vi "Main1.vi"(10 "Test Titel":string, 11 "Cluster 2":T1={"Test Titel"="", "Test Type "="", "Project Number"="NA", "Unit Family"="Package", "Test Procedure #"="", "Data Collection Rate (HZ)"="", "Cluster"={" Pressure /Torque/ LVDT"={"Boolean"=FALSE, "Boolean 2"=FALSE, "Boolean 3"=FALSE, "Boolean 4"=FALSE, "Boolean 5"=FALSE, "Boolean 6"=FALSE, "Boolean 7"=FALSE, "Boolean 8"=FALSE}, "Name of Channel"={"ch1"="", "ch1 2"="", "ch1 3"="", "ch1 4"="", "ch1 5"="", "ch1 6"="", "ch1 7"="", "ch1 8"=""}, "Create New Test"=FALSE, "Name of Channel 2"={"ch1"="", "ch1 2"="", "ch1 3"="", "ch1 4"="", "ch1 5"="", "ch1 6"="", "ch1 7"="", "ch1 8"="", "ch1 9"="", "ch1 10"="", "ch1 11"="", "ch1 12"="", "ch1 13"="", "ch1 14"="", "ch1 15"=""}, "MOD1 ThermoCouple"={"Boolean"=FALSE, "Boolean 2"=FALSE, "Boolean 3"=FALSE, "Boolean 4"=FALSE, "Boolean 5"=FALSE, "Boolean 6"=FALSE, "Boolean 7"=FALSE, "Boolean 8"=FALSE, "Boolean 9"=FALSE, "Boolean 10"=FALSE, "Boolean 11"=FALSE, "Boolean 12"=FALSE, "Boolean 13"=FALSE, "Boolean 14"=FALSE, "Boolean 15"=FALSE, "Boolean 16"=FALSE}, "Internal SFI sensor number"={"ch1"="", "ch1 2"="", "ch1 3"="", "ch1 4"="", "ch1 5"="", "ch1 6"="", "ch1 7"="", "ch1 8"=""}, "Internal SFI sensor number"={"ch1"="", "ch1 2"="", "ch1 3"="", "ch1 4"="", "ch1 5"="", "ch1 6"="", "ch1 7"="", "ch1 8"="", "ch1 9"="", "ch1 10"="", "ch1 11"="", "ch1 12"="", "ch1 13"="", "ch1 14"="", "ch1 15"=""}}, "Sensor Serial Num"="", "Calibration Due"=""}) -> (3 "Waveform Graph":dbl[][](graph))   [LabVIEW 2024]
uses:
  States.ctl
  Global 1.vi
  Wave forms.vi
panel:
  out "appended array 3":dbl[](array[numeric])
  in  "Table Control":string[][](table)
  out "Symbol":string
  in  "Combo Box":string(combo)
  in  "Boolean 2":bool
  in  "Log Interval\n(seconds)":dbl=0.5 min=0.1 max=10.0 step=0.1
  in  "Hours to Show 2":dbl=0.05
  in  "stop":bool
  out "appended array":string[](array[string])
  out "Array 3":string[](array[string])
  out "Array 2":string[](array[string])
  in  "Array":dbl[](array[numeric])
  in  "Boolean":bool
  out "Last Event Time (sec)":i32
  out "Event Counter":i32
  in  "Tab Control":enum32{"Main Configuration", "Graphs Display"}(tab)
  in  "End pro":bool
  in  "Settings Button":bool
  in  "Add paramter":bool
  in  "Select Parameter to ADD":string(combo)
  in  "Record Button":bool
  in  "end":bool caption="Pause Button 2"
  in  "Initial":bool caption="Pause Button"
  in  "Start Test":bool caption="OK Button"
  # "Valves Testing System"
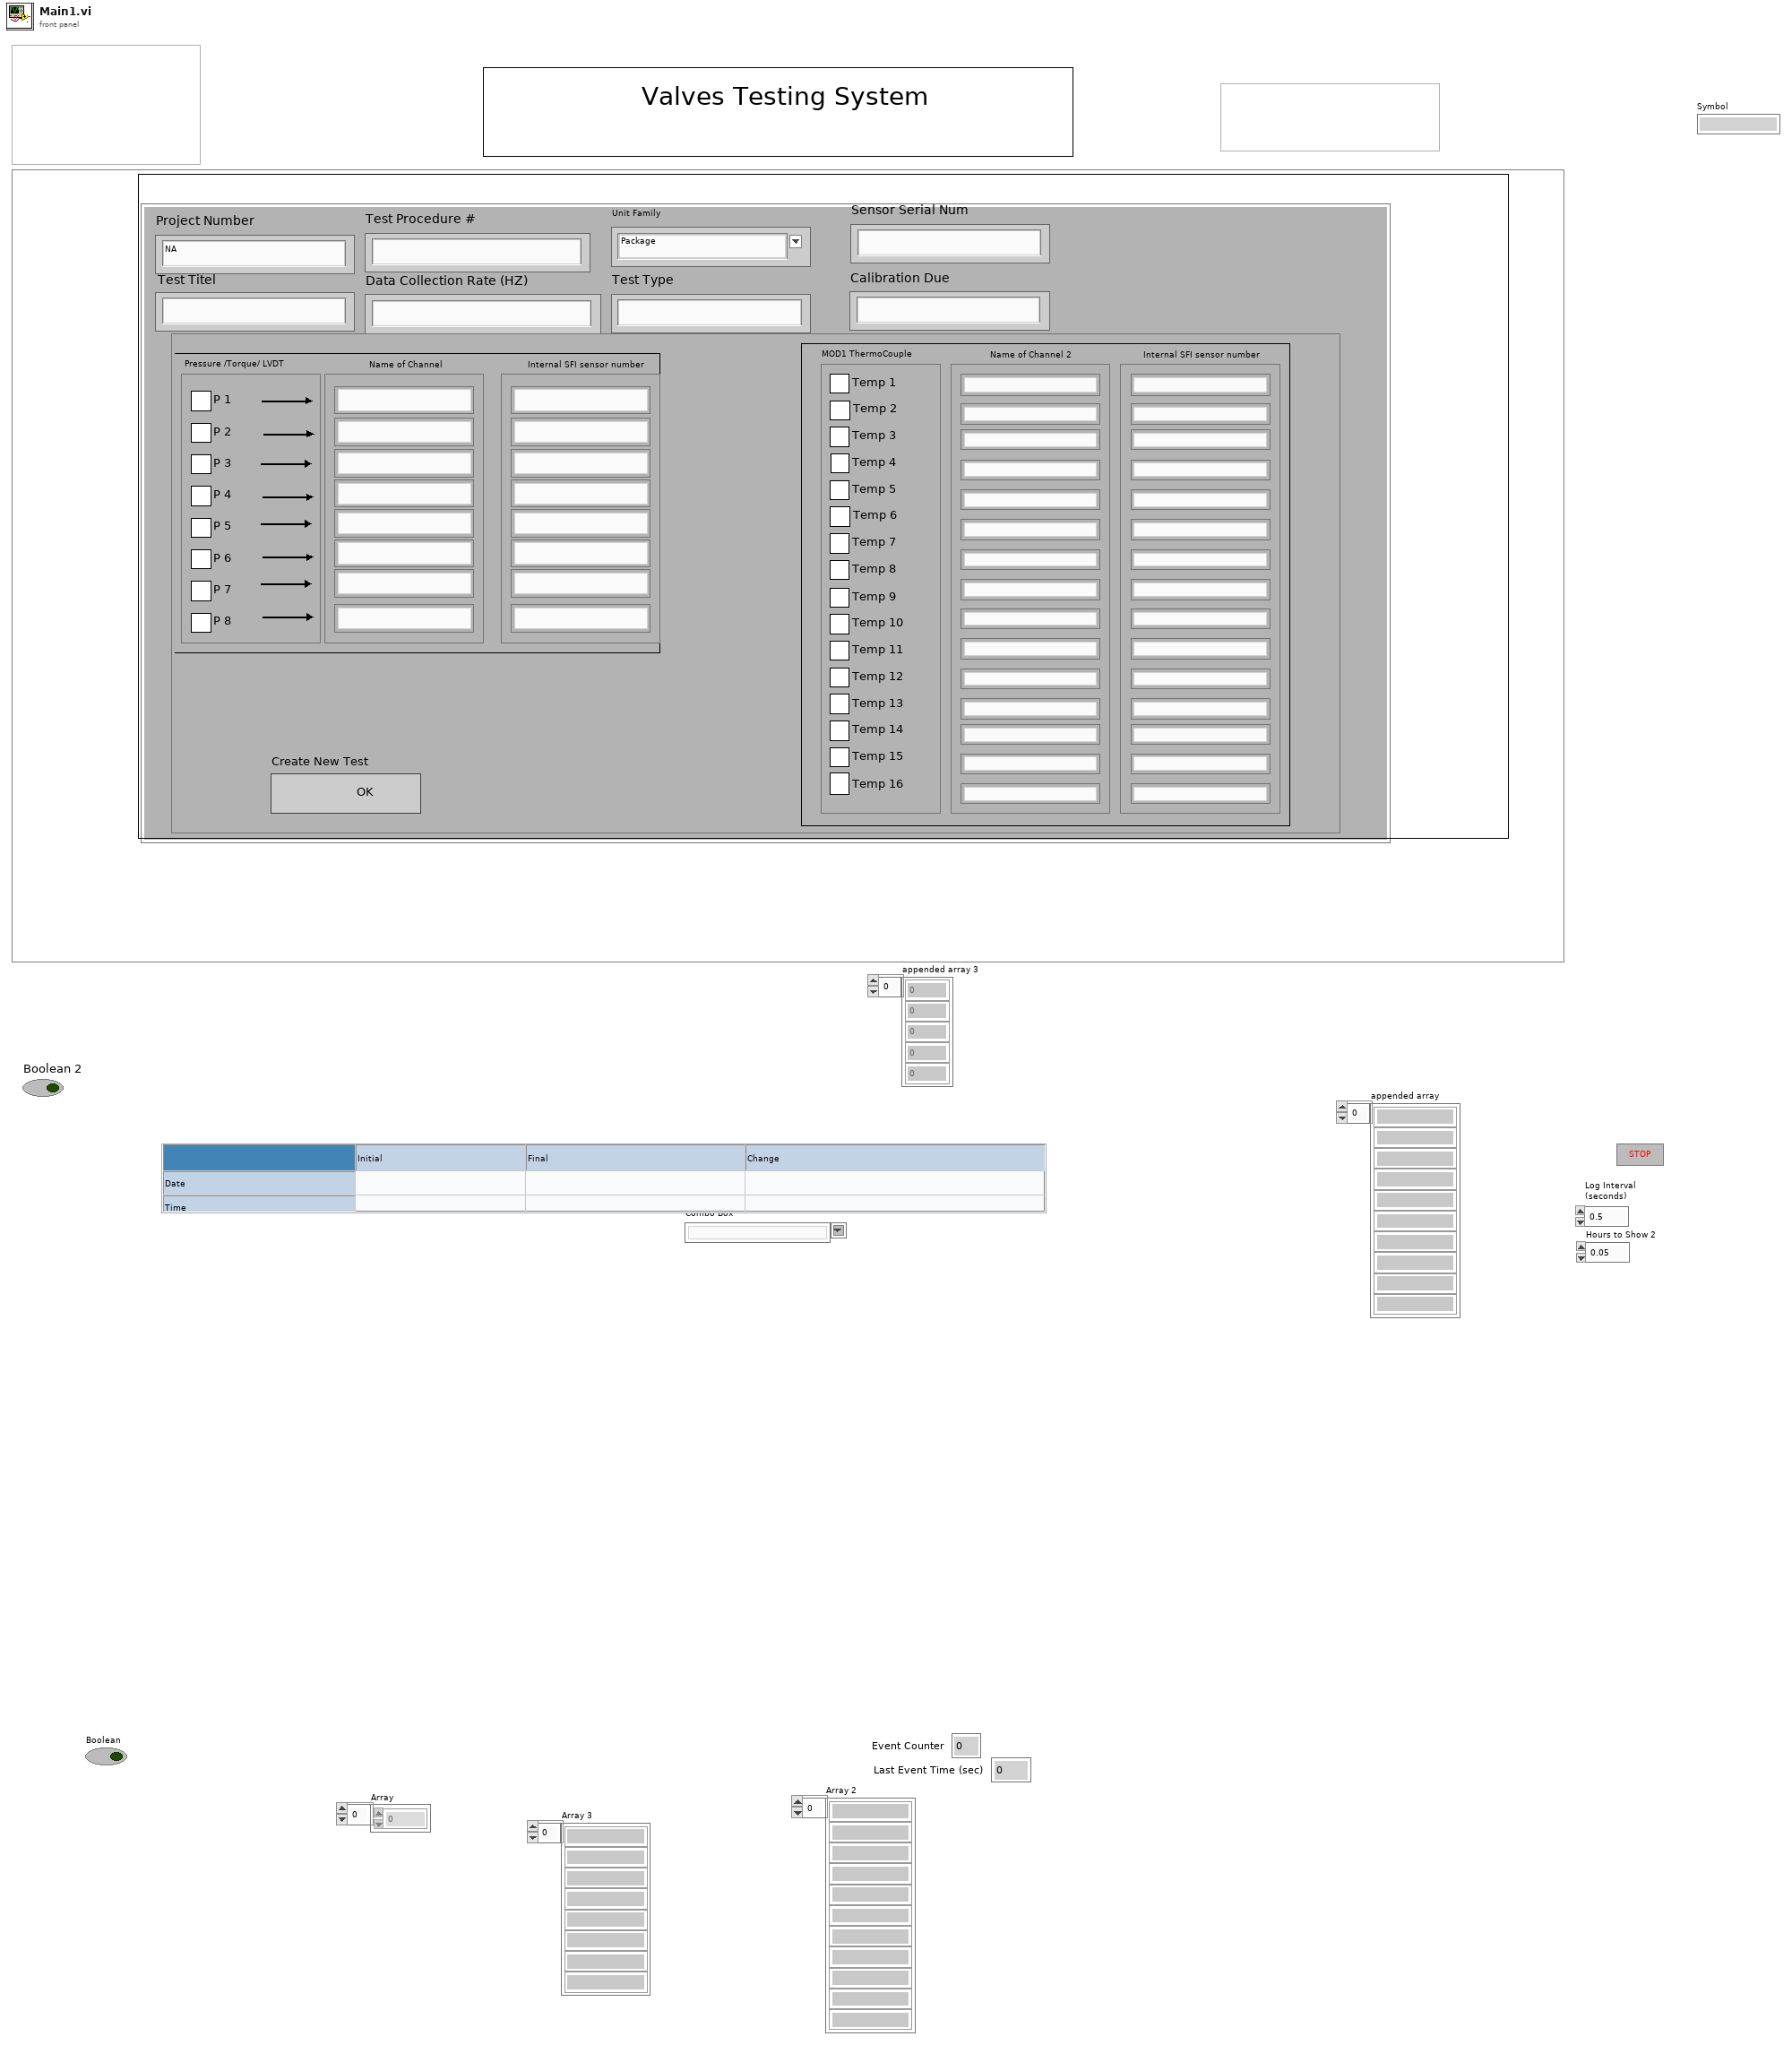
[diagram p1: front panel]
types:
  T1 = cluster{"Test Titel":string, "Test Type ":string, "Project Number":string, "Unit Family":string, "Test Procedure #":string, "Data Collection Rate (HZ)":string, "Cluster":cluster{" Pressure /Torque/ LVDT":cluster{"Boolean":bool, "Boolean 2":bool, "Boolean 3":bool, "Boolean 4":bool, "Boolean 5":bool, "Boolean 6":bool, "Boolean 7":bool, "Boolean 8":bool}, "Name of Channel":cluster{"ch1":string, "ch1 2":string, "ch1 3":string, "ch1 4":string, "ch1 5":string, "ch1 6":string, "ch1 7":string, "ch1 8":string}, "Create New Test":bool, "Name of Channel 2":cluster{"ch1":string, "ch1 2":string, "ch1 3":string, "ch1 4":string, "ch1 5":string, "ch1 6":string, "ch1 7":string, "ch1 8":string, "ch1 9":string, "ch1 10":string, "ch1 11":string, "ch1 12":string, "ch1 13":string, "ch1 14":string, "ch1 15":string}, "MOD1 ThermoCouple":cluster{"Boolean":bool, "Boolean 2":bool, "Boolean 3":bool, "Boolean 4":bool, "Boolean 5":bool, "Boolean 6":bool, "Boolean 7":bool, "Boolean 8":bool, "Boolean 9":bool, "Boolean 10":bool, "Boolean 11":bool, "Boolean 12":bool, "Boolean 13":bool, "Boolean 14":bool, "Boolean 15":bool, "Boolean 16":bool}, "Internal SFI sensor number":cluster{"ch1":string, "ch1 2":string, "ch1 3":string, "ch1 4":string, "ch1 5":string, "ch1 6":string, "ch1 7":string, "ch1 8":string}, "Internal SFI sensor number":cluster{"ch1":string, "ch1 2":string, "ch1 3":string, "ch1 4":string, "ch1 5":string, "ch1 6":string, "ch1 7":string, "ch1 8":string, "ch1 9":string, "ch1 10":string, "ch1 11":string, "ch1 12":string, "ch1 13":string, "ch1 14":string, "ch1 15":string}}, "Sensor Serial Num":string, "Calibration Due":string}
  T2 = typedef "States.ctl" = enum16{"Idel", "end test", "Selection", "Inittialize"}
  T3 = cluster{"Paramter":string, "Intital ":string, "Final":string, "Change":string, "Alarm Activate ":bool, "Symbol":string, "Value":string, "Alarm":bool}[]
  T4 = cluster{"Paramter":string, "Rate of Change":dbl, "X (sec)":dbl}[]
  T5 = cluster{"Paramter":string, "Intital ":string, "Final":string, "Change":string, "Alarm Activate ":bool, "Symbol":string, "Value":string, "Alarm":bool}
  T6 = cluster{"ch1":string, "ch1 2":string, "ch1 3":string, "ch1 4":string, "ch1 5":string, "ch1 6":string, "ch1 7":string, "ch1 8":string, "ch1 9":string, "ch1 10":string, "ch1 11":string, "ch1 12":string, "ch1 13":string, "ch1 14":string, "ch1 15":string}
  T7 = cluster{"Boolean":bool, "Boolean 2":bool, "Boolean 3":bool, "Boolean 4":bool, "Boolean 5":bool, "Boolean 6":bool, "Boolean 7":bool, "Boolean 8":bool, "Boolean 9":bool, "Boolean 10":bool, "Boolean 11":bool, "Boolean 12":bool, "Boolean 13":bool, "Boolean 14":bool, "Boolean 15":bool, "Boolean 16":bool}
  T8 = cluster{"Boolean":bool, "Boolean 2":bool, "Boolean 3":bool, "Boolean 4":bool, "Boolean 5":bool, "Boolean 6":bool, "Boolean 7":bool, "Boolean 8":bool}
  T9 = cluster{"ch1":string, "ch1 2":string, "ch1 3":string, "ch1 4":string, "ch1 5":string, "ch1 6":string, "ch1 7":string, "ch1 8":string}
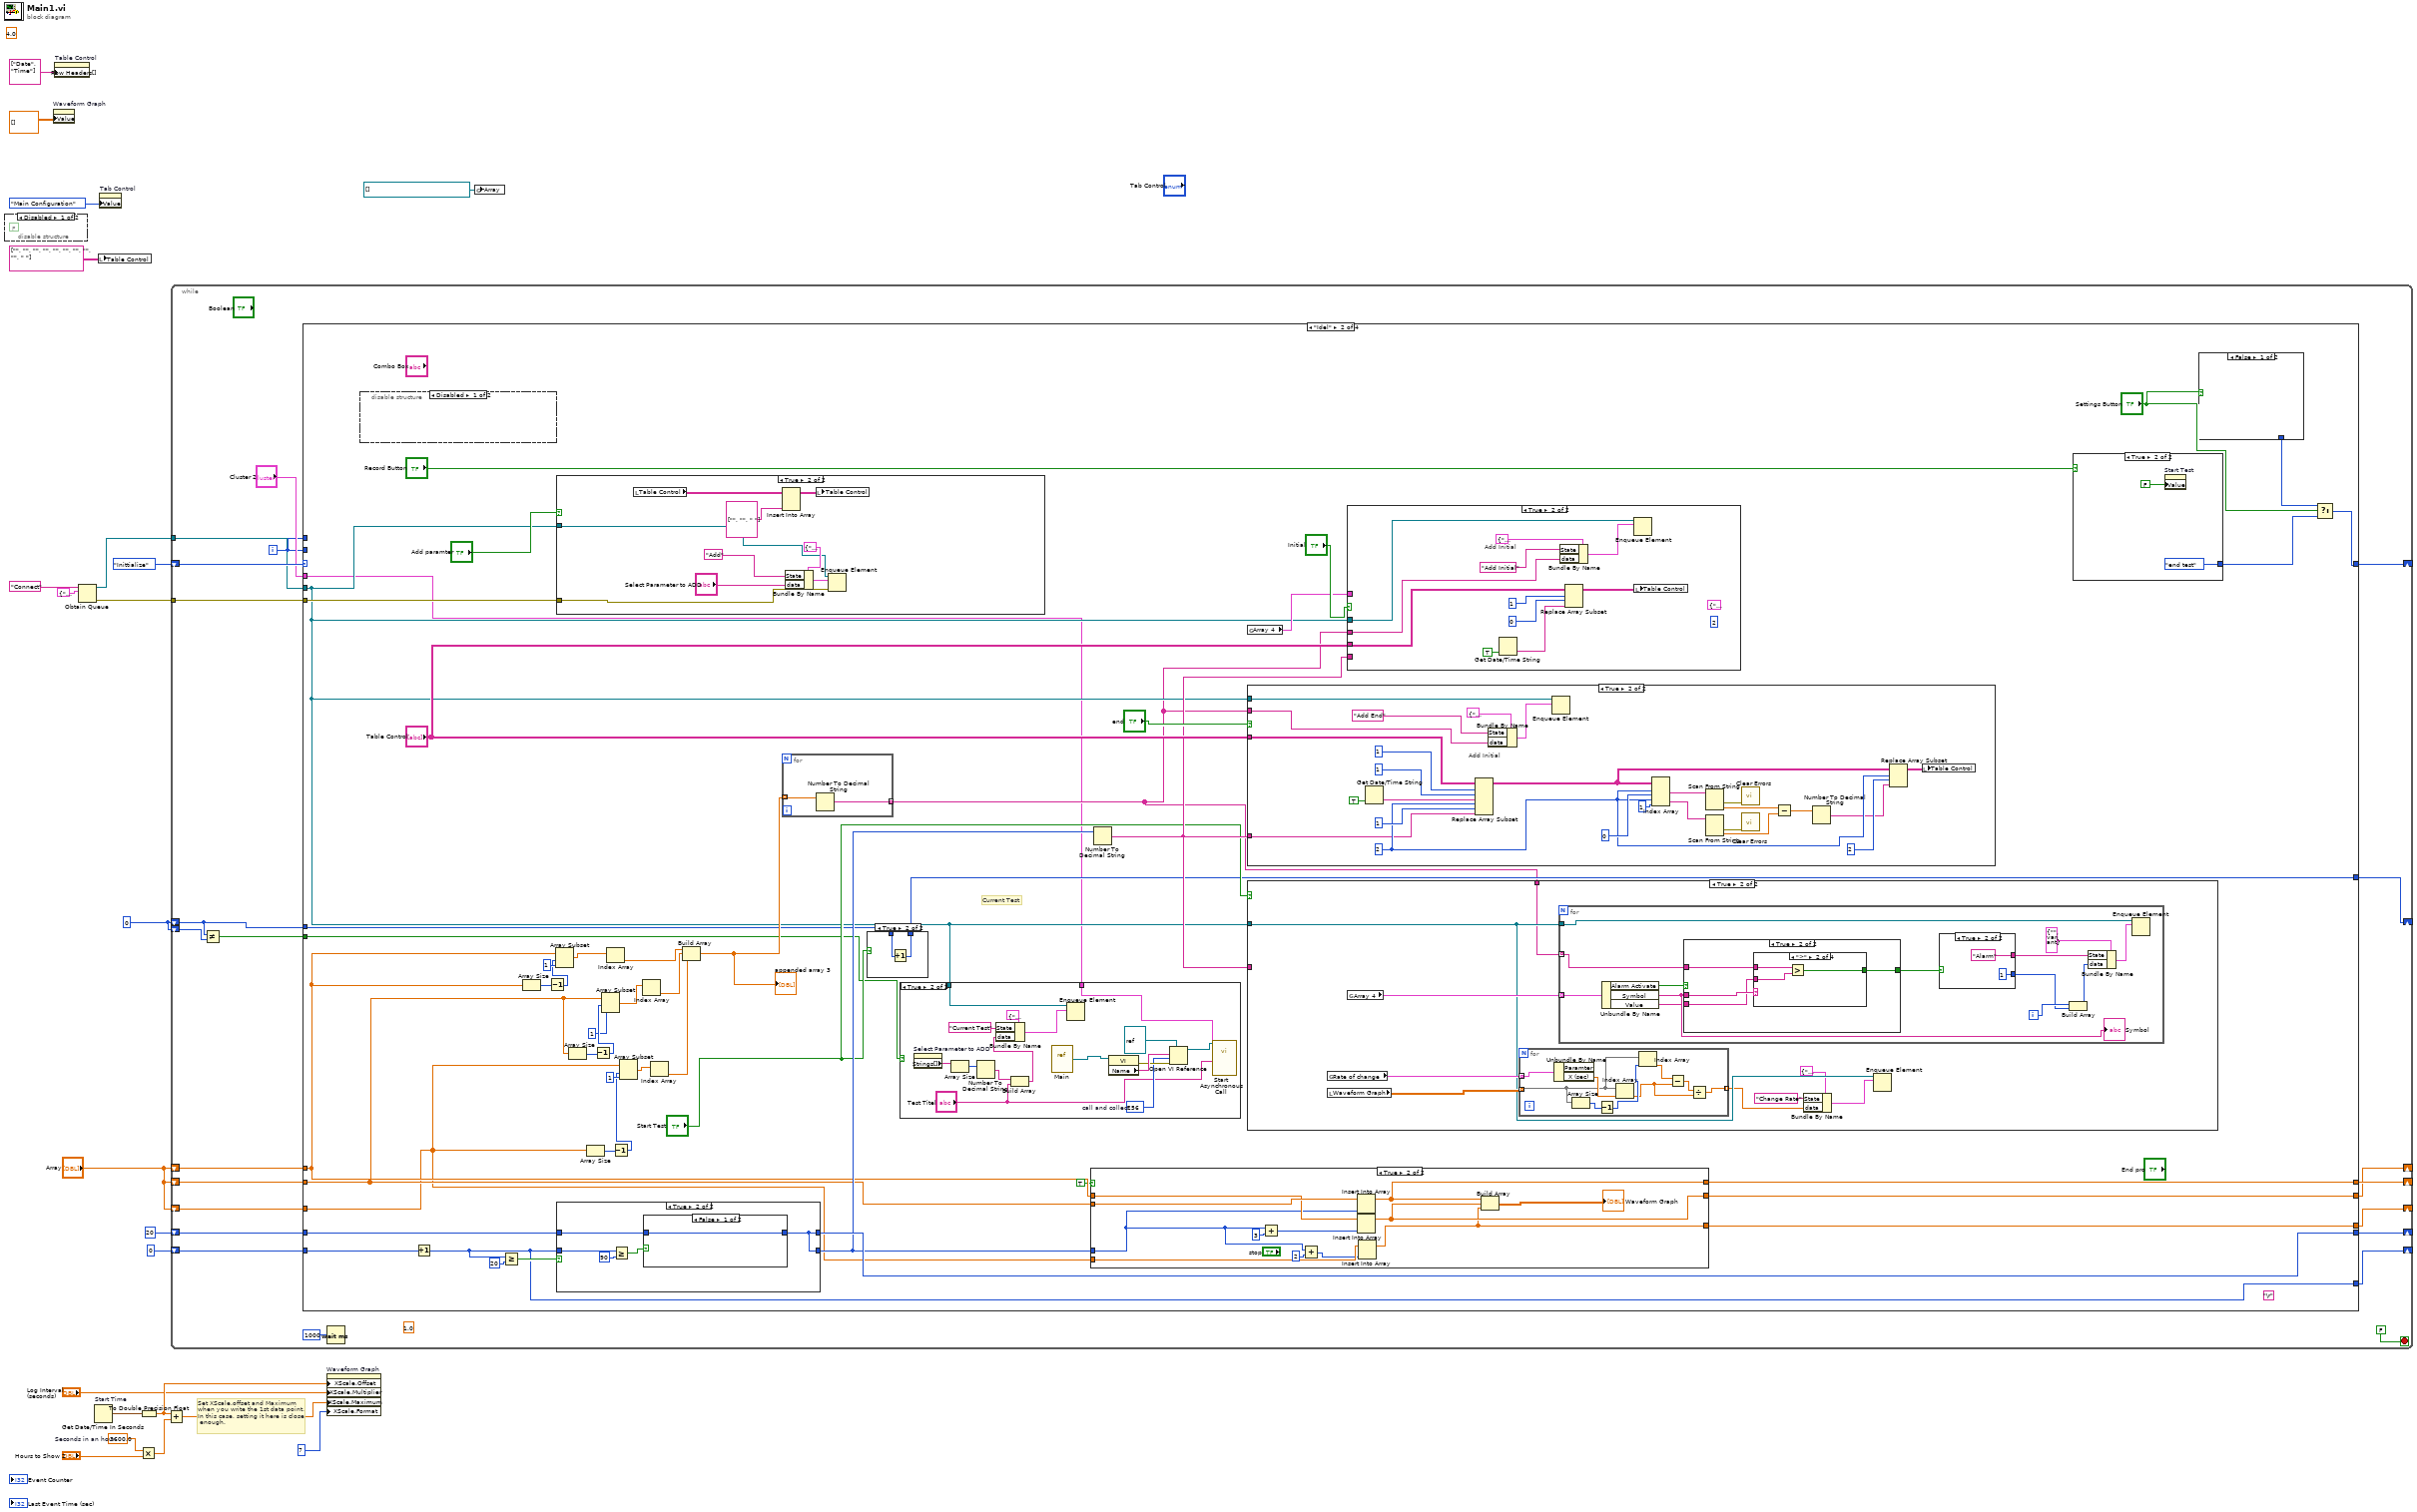
[diagram p0: block diagram]
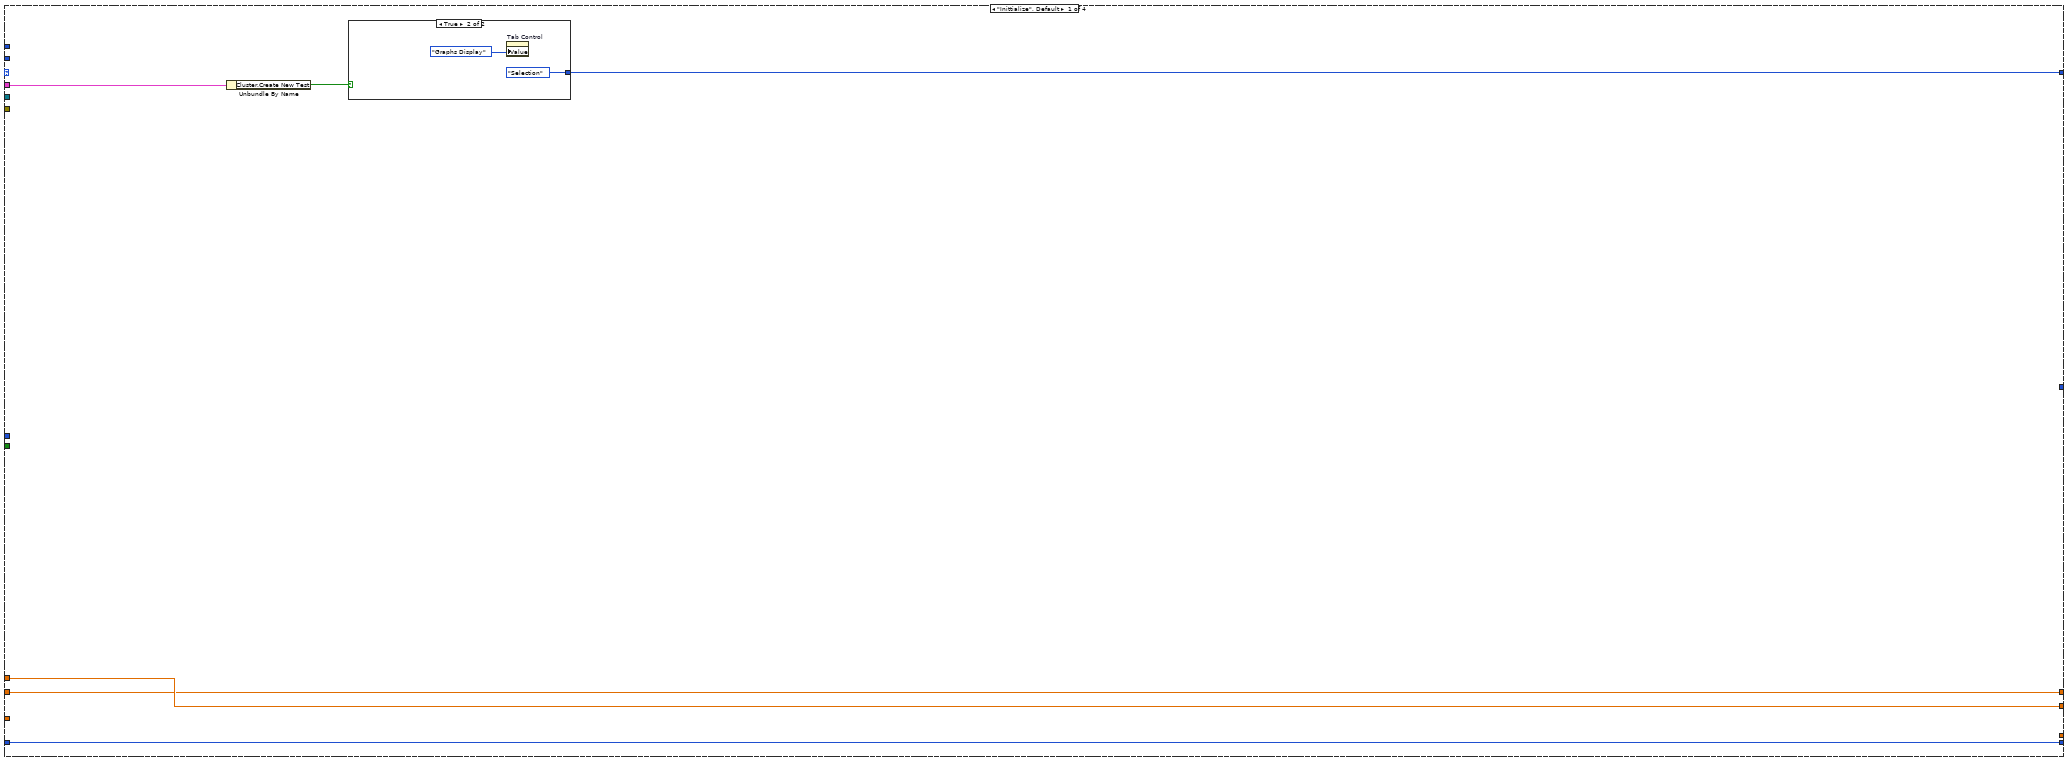
[diagram p3: hidden frame]
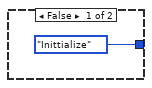
[diagram p4: hidden frame]
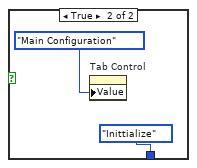
[diagram p7: hidden frame]
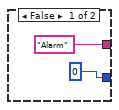
[diagram p9: hidden frame]
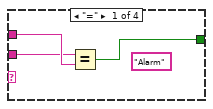
[diagram p11: hidden frame]
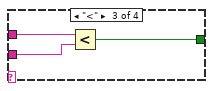
[diagram p12: hidden frame]
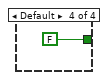
[diagram p13: hidden frame]
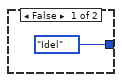
[diagram p15: hidden frame]
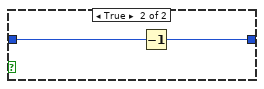
[diagram p20: hidden frame]
diagram:
  w2 = 0
  (unwired) 4.0
  w18 = 3600.0  # Seconds in an hour
  # "Set XScale.offset and Maximum\nwhen you write the 1st data point. \nIn this case, setting it here is close\n enough."
  n1 = disable-structure shown="Disabled" {
    frame Disabled {
      (unwired) FALSE ("OK Button")
    }
    frame Enabled {
    }
  }
  n2 = property on="Waveform Graph" class="WFGraph (strict)"("Value"=dbl[][] [] ("Waveform Graph")) -> ()  [unwired: 2 in, 2 out]
  n3 = property on="Table Control" class="Tbl (strict)"("Row Headers[]"=string[] ["Date", "Time"] ("Row Header Strings[]")) -> ()  [unwired: 2 in, 2 out]
  n4 = Obtain Queue(name (unnamed)="Connect", element data type=cluster{"State":string, "data":variant} {"State"="", "data"=variant}) -> (queue out=w5:refnum<queue>, error out=w4:errorcluster)  [unwired: 3 in, 1 out]
  n5 = Get Date/Time In Seconds "Start Time"() -> (seconds since 1Jan1904=w19:timestamp)
  n6 = local write "Table Control"(string[][] [["", "", "", "", ""], ["", "", "", "", " "]] ("Test Results")) -> ()
  n7 = property on="Tab Control" class="TabCtl (strict)"("Value"=enum32{"Main Configuration", "Graphs Display"}."Main Configuration" ("Tab Control")) -> ()  [unwired: 2 in, 2 out]
  n8 = Multiply(x=w18, y="Hours to Show 2") -> (x*y=w20:dbl)
  n9 = To Double Precision Float(number=w19) -> (double precision float=w13:dbl)
  n10 = Add(x=w13, y=w20) -> (x+y=w11:dbl)
  n11 = while {
    shift-right: [w41] -> _
    shift-left: States."Inittialize" -> [w44]
    shift-right: [w38] -> _
    shift-left: "Array" -> [w39]
    shift-right: [w32] -> _
    shift-left: 20 -> [w36]
    shift-right: [w34] -> _
    shift-left: "Array" -> [w35]
    shift-right: [w31] -> _
    shift-left: 0 -> [w33]
    tunnel: w5 -> [w30]
    tunnel: w4 -> [w29]
    shift-right: [w27] -> _
    shift-left: "Array" -> [w28]
    shift-right: [w23] -> _
    shift-left: w2 -> [w25]
    shift-left: w2 -> [w26]
    i -> [w37]
    stop <- FALSE stop-if-true
    (unwired) 1.0 ("Log Interval\n(seconds)")
    n12 = Not Equal?(x=w25, y=w26) -> (x != y?=w24:bool)
    n13 = case shown="\"Idel\"" w44 {
      tunnel: "Cluster 2" -> [w50 w54 w271 _]
      tunnel: [w47 w83 States."Idel" States."end test"] -> w41
      tunnel: w39 -> [w45 w70 _ _]
      tunnel: w37 -> [_ _ _ _]
      tunnel: [w45 w102 _ _] -> w38
      tunnel: w37 -> [_ _ _ _]
      tunnel: [w49 w98 w260 _] -> w32
      tunnel: w36 -> [w49 w97 w260 _]
      tunnel: w35 -> [w46 w79 _ _]
      tunnel: [w46 w91 _ _] -> w34
      tunnel: w33 -> [_ w90 _ _]
      tunnel: [_ w89 _ _] -> w31
      tunnel: w30 -> [_ w56 _ _]
      tunnel: w29 -> [_ w87 _ _]
      tunnel: w28 -> [_ w69 _ _]
      tunnel: [_ w81 _ _] -> w27
      tunnel: w25 -> [_ w60 _ _]
      tunnel: w24 -> [_ w59 _ _]
      tunnel: [_ w58 _ _] -> w23
      frame "Inittialize", Default {
        n14 = Unbundle By Name(w50) -> ("Cluster.Create New Test"=w48:bool)
        n15 = case shown="True" w48 {
          tunnel: [States."Inittialize" States."Selection"] -> w47
          frame False {
          }
          frame True {
            n16 = property on="Tab Control" class="TabCtl (strict)"("Value"=enum32{"Main Configuration", "Graphs Display"}."Graphs Display" ("Tab Control")) -> ()  [unwired: 2 in, 2 out]
          }
        }
      }
      frame "Idel" {
        (unwired) "\r"
        # "Current Test"
        n17 = disable-structure shown="Disabled" {
          frame Disabled {
          }
          frame Enabled {
          }
        }
        n18 = Increment(x=w90) -> (x+1=w89:i32)
        n19 = Greater Or Equal?(x=w89, y=20) -> (x >= y?=w99:bool)
        n20 = Array Size(array=w79) -> (size(s)=w78:i32)
        n21 = Decrement(x=w78) -> (x-1=w77:i32)
        n22 = Array Subset(array=w79, index=w77, length=1) -> (w68:dbl[])
        n23 = case shown="True" "Add paramter" {
          tunnel: w56 -> [_ w241]
          tunnel: w87 -> [_ w240]
          frame False {
          }
          frame True {
            n24 = local read "Table Control"() -> (w247:string[][])
            n25 = Insert Into Array(array=w247, new element=string[] ["", "", " "] ("new element/subarray")) -> (w246:string[][])  [unwired: 2 in]
            n26 = Bundle By Name(cluster=cluster{"State":string, "data":variant} {"State"="", "data"=variant}, "State"="Add", "data"="Select Parameter to ADD") -> (w244:cluster{"State":string, "data":variant})
            n27 = local write "Table Control"(w246) -> ()
            n28 = Enqueue Element(queue=w241, element=w244, error in (no error)=w240) -> ()  [unwired: 1 in, 3 out]
          }
        }
        n29 = case shown="True" w99 {
          tunnel: [w231 w235] -> w93
          tunnel: w89 -> [w231 w234]
          tunnel: [w230 w235] -> w98
          tunnel: w97 -> [w230 w236]
          frame False {
          }
          frame True {
            n30 = Greater Or Equal?(x=w234, y=90) -> (x >= y?=w232:bool)
            n31 = case shown="False" w232 {
              tunnel: w236 -> [w237 w239]
              tunnel: [w237 w238] -> w235
              frame False {
              }
              frame True {
                n32 = Decrement(x=w239) -> (x-1=w238:i32)
              }
            }
          }
        }
        n33 = Array Size(array=w70) -> (size(s)=w75:i32)
        n34 = Array Size(array=w69) -> (size(s)=w72:i32)
        n35 = Decrement(x=w75) -> (x-1=w76:i32)
        n36 = Array Subset(array=w70, index=w76, length=1) -> (w67:dbl[])
        n37 = Index Array(array=w68) -> (element=w65:dbl)  [unwired: 1 in]
        n38 = Decrement(x=w72) -> (x-1=w71:i32)
        n39 = Array Subset(array=w69, index=w71, length=1) -> (w66:dbl[])
        n40 = Index Array(array=w67) -> (element=w64:dbl)  [unwired: 1 in]
        n41 = Index Array(array=w66) -> (element=w63:dbl)  [unwired: 1 in]
        n42 = Build Array(w65, w64, w63) -> (w62:dbl[])
        "appended array 3" <- w62
        n43 = for {
          tunnel: w62 -> [w125] mode=indexing
          tunnel: [w124] -> w55 mode=indexing
          n44 = Number To Decimal String(number=w125) -> (decimal integer string=w124:string)  [unwired: 1 in]
        }
        n45 = case shown="True" "Start Test" {
          tunnel: w60 -> [w103 w105]
          tunnel: [w103 w104] -> w58
          frame False {
          }
          frame True {
            n46 = Increment(x=w105) -> (x+1=w104:i32)
          }
        }
        n47 = case shown="True" w59 {
          tunnel: w54 -> [_ w107]
          tunnel: w56 -> [_ w115]
          frame False {
          }
          frame True {
            w119 = 256  # call and collect
            n48 = property on="Select Parameter to ADD" class="CmbBox"() -> ("Strings[]"=w114:string[])  [unwired: 2 in, 2 out]
            n49 = Array Size(array=w114) -> (size(s)=w113:i32)
            n50 = Number To Decimal String(number=w113) -> (decimal integer string=w112:string)  [unwired: 1 in]
            n51 = Build Array(w112, "Test Titel") -> (w111:string[])
            n52 = Bundle By Name(cluster=cluster{"State":string, "data":variant} {"State"="", "data"=variant} ("input cluster"), "State"="Current Test", "data"=w111) -> (w118:cluster{"State":string, "data":variant})
            n53 = vi-ref "Main.vi"() -> (w106:refnum<vi>)
            n54 = Enqueue Element(queue=w115, element=w118) -> ()  [unwired: 2 in, 3 out]
            n55 = property class="VI"(reference=w106) -> (error out=w120:errorcluster, "Name"=w121:string)  [unwired: 1 in, 1 out]
            n56 = Open VI Reference(type specifier VI Refnum (for type only)=refnum<vi> refnum ("application reference (local)"), vi path=w121, options=w119, error in (no error)=w120) -> (vi reference=w109:refnum<vi>)  [unwired: 2 in, 1 out]
            n57 = call-by-ref "Start Asynchronous Call"(reference=w109, "Test Titel"="Test Titel", "Cluster 2"=w107) -> ()  [unwired: 10 in, 2 out]
          }
        }
        n58 = case shown="True" TRUE {
          tunnel: w70 -> [w217 w229]
          tunnel: [w217 w228] -> w102
          tunnel: w93 -> [_ w220]
          tunnel: w79 -> [w216 w226]
          tunnel: [w216 w224] -> w91
          tunnel: w69 -> [w215 w222]
          tunnel: [w215 w218] -> w81
          frame False {
          }
          frame True {
            n59 = Add(x=w220, y=3) -> (x+y=w225:i32)
            n60 = Add(x=w220, y=2) -> (x+y=w219:i32)
            n61 = Insert Into Array(array=w229, new element=w220) -> (w228:dbl[])  [unwired: 1 in]
            n62 = Insert Into Array(array=w226, new element=w225) -> (w224:dbl[])  [unwired: 1 in]
            n63 = Insert Into Array(array=w222, new element=w219) -> (w218:dbl[])  [unwired: 1 in]
            n64 = Build Array(w228, w224, w218) -> (→"Waveform Graph":dbl[][])
          }
        }
        n65 = Number To Decimal String(number=w93) -> (decimal integer string=w86:string)  [unwired: 1 in]
        n66 = global read "Global 1.vi" "Array 4"() -> (w88:T3)
        n67 = case shown="True" "end" {
          tunnel: "Table Control" -> [_ w202]
          tunnel: w86 -> [_ w179]
          tunnel: w56 -> [_ w183]
          tunnel: w55 -> [_ w178]
          frame False {
          }
          frame True {
            w189 = 2 ("index (row)")
            # "Add Initial"
            n68 = Get Date/Time String(want seconds? (F)=TRUE ("UTC format")) -> (time string=w199:string)  [unwired: 2 in, 1 out]
            n69 = Replace Array Subset(array=w202, new element #1=w199, index (row) #1=1 ("index (row)"), index (col) #1=1 ("disabled index (col)"), new element #2=w179, index (row) #2=w189, index (col) #2=1 ("disabled index (col)")) -> (w191:string[][])
            n70 = Bundle By Name(cluster=cluster{"State":string, "data":variant} {"State"="", "data"=variant}, "State"="Add End", "data"=w178) -> (w180:cluster{"State":string, "data":variant})
            n71 = Enqueue Element(queue=w183, element=w180) -> ()  [unwired: 2 in, 3 out]
            n72 = Index Array(array=w191, index (row) #1=w189, index (col) #1=0 ("disabled index (col)"), index (row) #2=w189, index (col) #2=1 ("index (col)")) -> (element #1=w195:string, element #2=w194:string)
            n73 = Scan From String(input string=w195) -> (error out=w185:errorcluster, output 1=w193:dbl)  [unwired: 4 in, 2 out]
            n74 = Scan From String(input string=w194) -> (error out=w184:errorcluster, output 1=w192:dbl)  [unwired: 4 in, 2 out]
            n75 = call <vilib>:"Clear Errors.vi"("error in (no error)"=w185) -> ()  [unwired: 5 in, 2 out]
            n76 = call <vilib>:"Clear Errors.vi"("error in (no error)"=w184) -> ()  [unwired: 5 in, 2 out]
            n77 = Subtract(x=w193, y=w192) -> (x-y=w187:dbl)
            n78 = Number To Decimal String(number=w187) -> (decimal integer string=w186:string)  [unwired: 1 in]
            n79 = Replace Array Subset(array=w191, new element=w186, index (row)=w189, index (col)=2 ("disabled index (col)")) -> (w190:string[][])
            n80 = local write "Table Control"(w190) -> ()
          }
        }
        n81 = case shown="True" "Start Test" {
          tunnel: w86 -> [_ _]
          tunnel: w56 -> [_ w131]
          tunnel: w55 -> [_ w126]
          frame False {
          }
          frame True {
            n82 = global read "Global 1.vi" "Rate of change"() -> (w133:T4)
            n83 = local read "Waveform Graph"() -> (w132:dbl[][])
            n84 = global read "Global 1.vi" "Array 4"() -> (w134:T3)
            n85 = for {
              tunnel: w133 -> [w143] mode=indexing
              tunnel: w132 -> [w141] mode=indexing
              tunnel: [w135] -> w128 mode=indexing
              n86 = Unbundle By Name(w143) -> ("X (sec)"=w142:dbl)  [unwired: 1 out]
              n87 = Array Size(array=w141) -> (size(s)=w140:i32)
              n88 = Decrement(x=w140) -> (x-1=w139:i32)
              n89 = Index Array(array=w141, index=w142) -> (element=w136:dbl)
              n90 = Index Array(array=w141, index=w139) -> (element=w138:dbl)
              n91 = Subtract(x=w138, y=w136) -> (x-y=w137:dbl)
              n92 = Divide(x=w137, y=w136) -> (x/y=w135:dbl)
            }
            n93 = for {
              tunnel: w134 -> [w156] mode=indexing
              tunnel: w131 -> [w150]
              tunnel: w126 -> [w147] mode=indexing
              i -> [w146]
              n94 = Unbundle By Name(w156) -> ("Alarm Activate"=w155:bool, "Symbol"=w154:string, "Value"=w153:string)
              "Symbol" <- w154
              n95 = case shown="True" w155 {
                tunnel: w154 -> [_ w164]
                tunnel: w153 -> [_ w163]
                tunnel: w147 -> [_ w162]
                tunnel: [_ w161] -> w151
                frame False {
                }
                frame True {
                  n96 = case shown="\">\"" w164 {
                    tunnel: w163 -> [w166 w168 w171 _]
                    tunnel: w162 -> [w167 w169 w172 _]
                    tunnel: [w165 w170 w173 FALSE] -> w161
                    frame "=" {
                      (unwired) "Alarm" ("State")
                      n97 = Equal?(x=w166, y=w167) -> (x = y?=w165:bool)
                    }
                    frame ">" {
                      n98 = Greater?(x=w169, y=w168) -> (0:w170:bool)
                    }
                    frame "<" {
                      n99 = Less?(x=w172, y=w171) -> (x < y?=w173:bool)
                    }
                    frame Default {
                    }
                  }
                }
              }
              n100 = case shown="True" w151 {
                tunnel: ["Alarm" ("State") "Alarm" ("State")] -> w152
                tunnel: [0 ("Numeric") 1 ("Numeric")] -> w145
                frame False {
                }
                frame True {
                }
              }
              n101 = Build Array(w146, w145) -> (w144:i32[])
              n102 = Bundle By Name(cluster=cluster{"State":string, "data":variant} {"State"="", "data"=variant} ("element"), "State"=w152, "data"=w144) -> (w148:cluster{"State":string, "data":variant})
              n103 = Enqueue Element(queue=w150, element=w148) -> ()  [unwired: 2 in, 3 out]
            }
            n104 = Bundle By Name(cluster=cluster{"State":string, "data":variant} {"State"="", "data"=variant} ("input cluster"), "State"="Change Rate", "data"=w128) -> (w127:cluster{"State":string, "data":variant})
            n105 = Enqueue Element(queue=w131, element=w127) -> ()  [unwired: 2 in, 3 out]
          }
        }
        n106 = case shown="True" "Initial" {
          tunnel: "Table Control" -> [_ w214]
          tunnel: w86 -> [_ _]
          tunnel: w88 -> [_ _]
          tunnel: w56 -> [_ w208]
          tunnel: w55 -> [_ w204]
          frame False {
          }
          frame True {
            (unwired) T5 {"Paramter"="", "Intital "="", "Final"="", "Change"="", "Alarm Activate "=FALSE, "Symbol"="", "Value"="", "Alarm"=FALSE} ("new element/subarray")
            (unwired) 2 ("index (row)")
            # "Add Initial"
            n107 = Get Date/Time String(want seconds? (F)=TRUE ("UTC format")) -> (time string=w209:string)  [unwired: 2 in, 1 out]
            n108 = Bundle By Name(cluster=cluster{"State":string, "data":variant} {"State"="", "data"=variant}, "State"="Add Initial", "data"=w204) -> (w206:cluster{"State":string, "data":variant})
            n109 = Replace Array Subset(array=w214, new element=w209, index (row)=1, index (col)=0 ("disabled index (col)")) -> (w212:string[][])
            n110 = Enqueue Element(queue=w208, element=w206) -> ()  [unwired: 2 in, 3 out]
            n111 = local write "Table Control"(w212) -> ()
          }
        }
        n112 = case shown="True" "Record Button" {
          tunnel: [States."Idel" States."end test"] -> w84
          frame False {
          }
          frame True {
            n113 = property on="Start Test" class="Bool"("Value"=FALSE ("OK Button")) -> ()  [unwired: 2 in, 2 out]
          }
        }
        n114 = case shown="False" "Settings Button" {
          tunnel: [_ States."Inittialize"] -> w82
          frame False {
          }
          frame True {
            n115 = property on="Tab Control" class="TabCtl (strict)"("Value"=enum32{"Main Configuration", "Graphs Display"}."Main Configuration" ("Tab Control")) -> ()  [unwired: 2 in, 2 out]
          }
        }
        n116 = Select(t=w82, s="Settings Button", f=w84) -> (s? t:f=w83:T2)
      }
      frame "Selection" {
        w262 = string[] []
        n117 = Unbundle By Name(w271) -> ("Cluster.Name of Channel 2"=w266:T6, "Cluster.MOD1 ThermoCouple"=w270:T7, "Cluster.Pressure /Torque/ LVDT"=w269:T8, "Cluster.Name of Channel"=w264:T9, "Project Number"=w253:string, "Test Type"=w251:string, "Unit Family"=w256:string, "Test Type"=w255:string, "Data Collection Rate (HZ)"=w254:string, "Sensor Serial Num"=w250:string)
        n118 = local read "Test Titel"() -> (w249:string)
        n119 = flat-sequence {
          tunnel: w261 -> [w277]
          frame #0 {
            n120 = for {
              N: 14 -> [_]
              i -> [w274]
              n121 = property on="Waveform Graph" class="WFGraph (strict)"("ActYScl"=w274, "YScale.Visible"=FALSE ("Y Scale.Visible")) -> ()  [unwired: 2 in, 2 out]
            }
          }
          frame #1 {
            n122 = Index Array(array=w277, index=0) -> (element=w275:string)
            n123 = flat-sequence {
              tunnel: w277 -> [w278]
              tunnel: w275 -> [w286]
              frame #0 {
                n124 = for {
                  tunnel: w278 -> [w281] mode=indexing
                  i -> [w280]
                  n125 = disable-structure shown="Enabled" {
                    disable-tunnel: w281 -> [w284 _]
                    disable-tunnel: w280 -> [w283 _]
                    disable-tunnel: TRUE ("Y Scale.Visible") -> [w282 _]
                    frame Enabled {
                      n126 = property on="Waveform Graph" class="WFGraph (strict)"("YScale.NameLbl.Text"=w284, "ActYScl"=w283, "YScale.Visible"=w282) -> ()  [unwired: 2 in, 2 out]
                    }
                    frame Disabled {
                    }
                  }
                }
              }
              frame #1 {
                n127 = property on="Waveform Graph" class="WFGraph (strict)"("YScale.NameLbl.Text"=w286, "ActYScl"=0 ("Active Y Scale")) -> ()  [unwired: 2 in, 2 out]
              }
            }
          }
        }
        n128 = Build Array(w253, w251, w256, w255, w254, w250, w249) -> (w252:string[])
        n129 = global write "Global 1.vi" "Initial"(w252) -> ()
        n130 = Cluster To Array(cluster=w270) -> (array=w268:bool[])
        n131 = Cluster To Array(cluster=w269) -> (array=w267:bool[])
        n132 = Cluster To Array(cluster=w264) -> (array=w263:string[])
        n133 = Cluster To Array(cluster=w266) -> (array=w265:string[])
        n134 = for {
          tunnel: w268 -> [w298] mode=indexing
          tunnel: w265 -> [w295] mode=indexing
          shift-right: [w296] -> w258
          shift-left: w262 -> [w297]
          n135 = case shown="True" w298 {
            tunnel: w297 -> [w299 w302]
            tunnel: [w299 w301] -> w296
            tunnel: w295 -> [_ w300]
            frame False {
            }
            frame True {
              n136 = Insert Into Array(array=w302, new element=w300) -> (w301:string[])  [unwired: 1 in]
            }
          }
        }
        "Array 2" <- w258
        n137 = for {
          tunnel: w267 -> [w290] mode=indexing
          tunnel: w263 -> [w289] mode=indexing
          shift-right: [w287] -> w259
          shift-left: w262 -> [w288]
          n138 = case shown="True" w290 {
            tunnel: w288 -> [w291 w294]
            tunnel: [w291 w293] -> w287
            tunnel: w289 -> [_ w292]
            frame False {
            }
            frame True {
              n139 = Insert Into Array(array=w294, new element=w292) -> (w293:string[])  [unwired: 1 in]
            }
          }
        }
        "Array 3" <- w259
        n140 = Build Array (concatenate)(w258, w259) -> (w261:string[])
        "appended array" <- w261
        n141 = property on="Select Parameter to ADD" class="CmbBox"("Strings[]"=w261) -> ()  [unwired: 2 in, 2 out]
      }
      frame "end test" {
        n142 = case shown="True" "Boolean 2" {
          frame False {
          }
          frame True {
          }
        }
      }
    }
    n143 = Wait (ms)(milliseconds to wait=u32 1000) -> ()  [unwired: 1 out]
  }
  n144 = property on="Waveform Graph" class="WFGraph (strict)"("XScale.Offset"=w13, "XScale.Multiplier"="Log Interval\n(seconds)", "XScale.Maximum"=w11, "XScale.Format"=u8 7 ("X Scale.Display Format:Format")) -> ()  [unwired: 2 in, 2 out]
  n145 = global write "Wave forms.vi" "Array"(refnum<vi>[] [] ("Array")) -> ()
